vi "Create AO Resource.vi"(8 "error in (no error)":errorcluster) -> (0 "error out":errorcluster, 2 "found?":bool, 3 "task out":i32)   [LabVIEW 2021]
uses:
  <userlib>/DAQNavi Polymorphic VI/create/DAQNavi Create Channel(AO-Voltage).vi
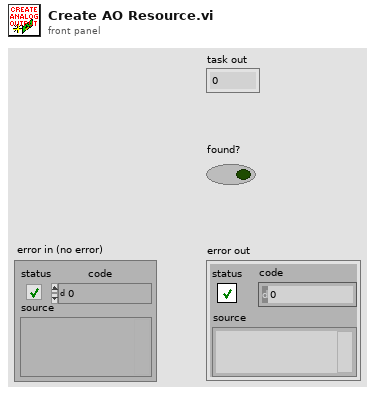
[diagram p1: front panel]
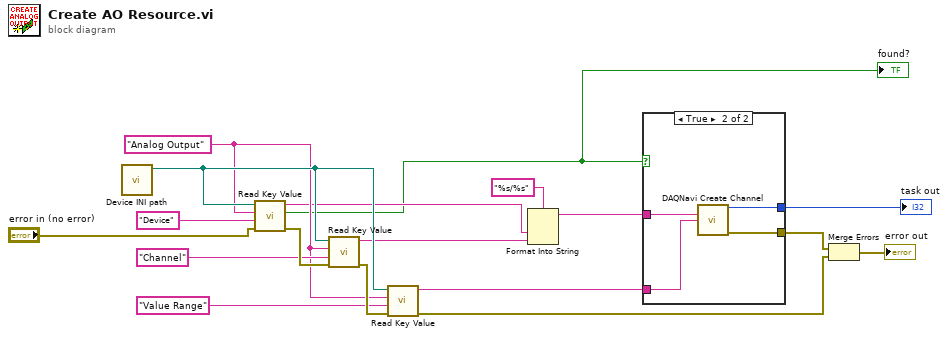
[diagram p0: block diagram]
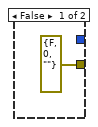
[diagram p2: hidden frame]
diagram:
  w13 = "Analog Output" ("Device Session Name")
  n1 = call "Device INI path.vi"() -> ("appended path"=w14:path)  [unwired: 11 in]
  n2 = call "Read Key Value.vi"("error in (no error)"="error in (no error)", "key"="Device" ("Search Key"), "Device Session Name"=w13, "appended path"=w14) -> ("error out"=w17:errorcluster, "found?"=w7:bool, "value"=w10:string)  [unwired: 5 in]
  "found?" <- w7
  n3 = call "Read Key Value.vi"("error in (no error)"=w17, "key"="Channel" ("Search Key"), "Device Session Name"=w13, "appended path"=w14) -> ("error out"=w15:errorcluster, "value"=w9:string)  [unwired: 5 in, 1 out]
  n4 = call "Read Key Value.vi"("error in (no error)"=w15, "key"="Value Range" ("Search Key"), "Device Session Name"=w13, "appended path"=w14) -> ("error out"=w1:errorcluster, "value"=w5:string)  [unwired: 5 in, 1 out]
  n5 = Format Into String(format string="%s/%s", w10, w9) -> (resulting string=w6:string)  [unwired: 2 in, 1 out]
  n6 = case shown="True" w7 {
    tunnel: [errorcluster {"status"=FALSE, "code"=0, "source"=""} ("error out") w23] -> w3
    tunnel: w6 -> [_ w22]
    tunnel: w5 -> [_ w21]
    tunnel: [_ w20] -> w4
    frame False {
    }
    frame True {
      n7 = call-poly <userlib>:"DAQNavi Create Channel.vi"("physical channels"=w22, "value range"=w21) -> ("task out"=w20:i32, "error out"=w23:errorcluster)  [unwired: 12 in]
    }
  }
  "task out" <- w4
  n8 = Merge Errors(w3, w1) -> (→"error out":errorcluster)
